vi "Manual.vi"() -> ()   [LabVIEW 2021]
uses:
  <vilib>/myRIO/Instrument Drivers/Onboard IO/DIO/typedefs/DIO Reference.ctl
  <vilib>/myRIO/Common/Instrument Driver Framework/Utilities/typedefs/myRIO Generic Hardware Reference.ctl
  <vilib>/myRIO/Common/Instrument Driver Framework/Utilities/typedefs/Hardware Version Enum.ctl
  <vilib>/myRIO/Common/Instrument Driver Framework/Utilities/typedefs/myRIO v1.0 Reference.ctl
  <vilib>/myRIO/Common/Instrument Driver Framework/Utilities/typedefs/Generic FPGA Reference.ctl
  <vilib>/myRIO/Common/Instrument Driver Framework/myRIO v1.0/DIO/typedefs/DIO Channels List.ctl
  <vilib>/myRIO/Common/Instrument Driver Framework/myRIO v1.0/DIO/typedefs/DIO Channels Enum.ctl
  <vilib>/userDefined/High Color/nirio_resource_hc.ctl
  <vilib>/myRIO/Instrument Drivers/Onboard IO/PWM/typedefs/PWM Reference.ctl
  <vilib>/myRIO/Common/Instrument Driver Framework/myRIO v1.0/PWM/typedefs/PWM Channels Enum.ctl
  <vilib>/myRIO/Instrument Drivers/Onboard IO/PWM/typedefs/PWM Configuration.ctl
  <vilib>/myRIO/Common/Instrument Driver Framework/Utilities/vis/Is FPGA Ref Available.vi
  <vilib>/myRIO/Common/Instrument Driver Framework/myRIO v1.0/DIO/vis/myRIO v1.1 Open DIO.vi
  <vilib>/myRIO/Instrument Drivers/Onboard IO/DIO/vis/Write.vi
  <vilib>/myRIO/Common/Instrument Driver Framework/myRIO v1.0/PWM/vis/myRIO v1.1 Open PWM.vi
  <vilib>/myRIO/Instrument Drivers/Onboard IO/PWM/vis/Set Duty Cycle and Frequency.vi
  <vilib>/myRIO/Common/Instrument Driver Framework/Utilities/vis/Validate Channels.vi
  <vilib>/myRIO/Common/Instrument Driver Framework/myRIO v1.0/DIO/vis/myRIO v1.0 Reserve DIO.vi
  <vilib>/myRIO/Common/Instrument Driver Framework/myRIO v1.0/PWM/vis/myRIO v1.0 Reserve PWM.vi
  <vilib>/myRIO/Common/Instrument Driver Framework/myRIO v1.0/Resource Manager/vis/myRIO v1.0 Reserve Channel List.vi
  <vilib>/myRIO/Common/Instrument Driver Framework/myRIO v1.0/DIO/vis/myRIO v1.0 Build MUX Configuration DIO.vi
  <vilib>/myRIO/Common/Instrument Driver Framework/myRIO v1.0/PWM/vis/myRIO v1.0 Build MUX Configuration PWM.vi
  <vilib>/myRIO/Common/Instrument Driver Framework/myRIO v1.0/Resource Manager/vis/myRIO v1.0 Reserve Channel.vi
  <vilib>/myRIO/Common/Instrument Driver Framework/myRIO v1.0/Resource Manager/vis/myRIO v1.0 Unreserve Channel.vi
  <vilib>/myRIO/Common/Instrument Driver Framework/myRIO v1.0/Resource Manager/vis/myRIO v1.0 Create Configuration List.vi
  <vilib>/myRIO/Common/Instrument Driver Framework/myRIO v1.0/Resource Manager/vis/myRIO v1.0 Build Mutex Name.vi
  <vilib>/Utility/VariantDataType/GetNumericInfo.vi
  <vilib>/Utility/error.llb/Error Cluster From Error Code.vi
  <vilib>/myRIO/Common/Instrument Driver Framework/myRIO v1.0/myRIO v1.1 Open.vi
  <vilib>/myRIO/Common/Instrument Driver Framework/Utilities/vis/IO Manager.vi
  <vilib>/myRIO/Common/Instrument Driver Framework/Utilities/vis/Configuration Manager.vi
  <vilib>/myRIO/Common/Instrument Driver Framework/myRIO v1.0/Resource Manager/vis/myRIO v1.0 Configure IO.vi
  <vilib>/myRIO/Common/Instrument Driver Framework/myRIO v1.0/myRIO v1.0 Close.vi
  <vilib>/myRIO/Common/Instrument Driver Framework/myRIO v1.0/DIO/vis/myRIO v1.0 Write DIO.vi
  <vilib>/myRIO/Common/Instrument Driver Framework/myRIO v1.0/PWM/vis/myRIO v1.0 Write PWM.vi
  <vilib>/myRIO/Express VI/Onboard IO/DO/DO Express VI.xnode
  <vilib>/myRIO/Instrument Drivers/Onboard IO/DIO/vis/myRIO DIO Open.xnode
  <vilib>/myRIO/Express VI/Onboard IO/PWM/PWM Express VI.xnode
  <vilib>/myRIO/Instrument Drivers/Onboard IO/PWM/vis/myRIO PWM Open.xnode
  <vilib>/myRIO/Instrument Drivers/Onboard IO/PWM/PWM.lvlib
  <vilib>/myRIO/Instrument Drivers/Onboard IO/DIO/DIO.lvlib
panel:
  out "Shoot Speed":dbl
  out "B":bool
  out "D":bool
  out "A":bool
  out "C":bool
  out "Robot Speed":dbl format="%#_1f"
  out "Joystick Status":bool
  out "Direction":dbl
  in  "stop":bool
  # "MOTOR ORIENTATION"
  # "MyRIO-SooYewGuan\n\n0.025\n0.125\n\n0.105\n0.125"
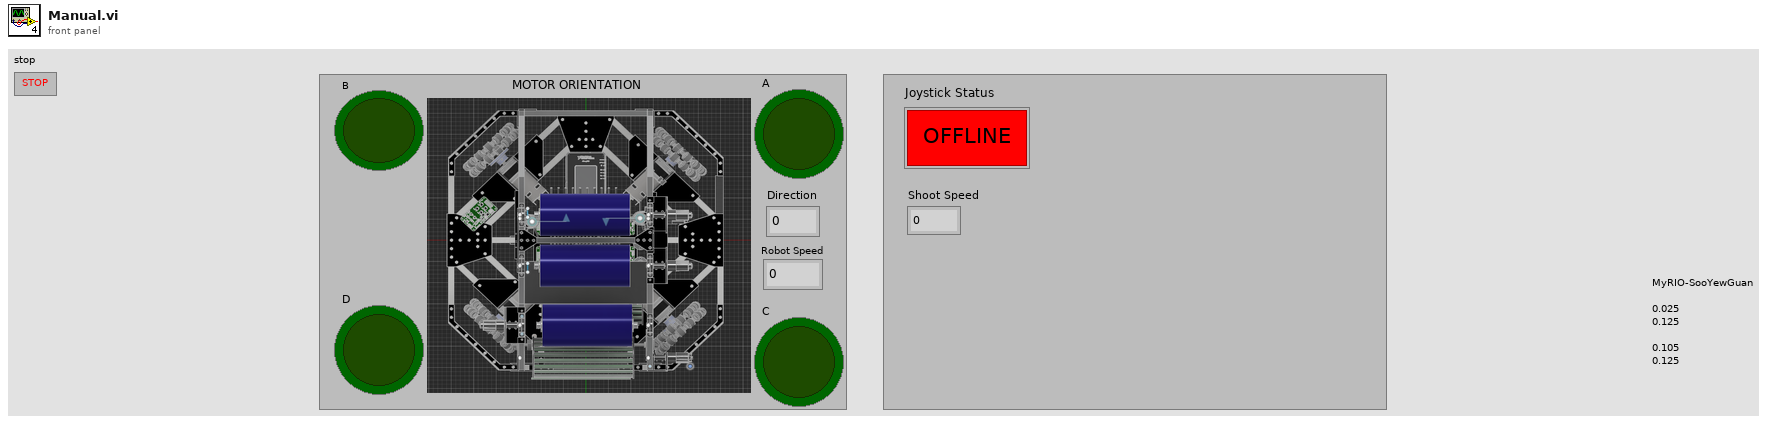
[diagram p1: front panel]
types:
  T1 = typedef "DIO.lvlib/DIO Reference.ctl" = cluster{"myRIO Reference":T2, "DIO Channels List":T6}
  T2 = typedef "myRIO Generic Hardware Reference.ctl" = cluster{"myRIO Model":T3, "myRIO Hardware Reference":T4}
  T3 = typedef "Hardware Version Enum.ctl" = enum16{"Unknown", "myRIO-1900", "myRIO-1950", "roboRIO", "NI ELVIS RIO CM", "ELVIS III"}
  T4 = typedef "myRIO v1.0 Reference.ctl" = cluster{"Generic FPGA Reference":T5, "Allow multiple opens":bool}
  T5 = typedef "Generic FPGA Reference.ctl" = refnum<k20>
  T6 = typedef "DIO Channels List.ctl" = T7[]
  T7 = typedef "DIO Channels Enum.ctl" = enum16{"Not Connected", "C/DIO0", "C/DIO1", "C/DIO2", "C/DIO3", "C/DIO4", "C/DIO5", "C/DIO6", "C/DIO7", "A/DIO0", "A/DIO1", "A/DIO2", "A/DIO3", "A/DIO4", "A/DIO5", "A/DIO6", "A/DIO7", "A/DIO8", "A/DIO9", "A/DIO10", "A/DIO11", "A/DIO12", "A/DIO13", "A/DIO14", "A/DIO15", "A/DIO16", "A/DIO17", "A/DIO18", "A/DIO19", "B/DIO0", "B/DIO1", "B/DIO2", "B/DIO3", "B/DIO4", "B/DIO5", "B/DIO6", "B/DIO7", "B/DIO8", "B/DIO9", "B/DIO10", "B/DIO11", "B/DIO12", "B/DIO13", "B/DIO14", "B/DIO15", "B/DIO16", "B/DIO17", "B/DIO18", "B/DIO19", "LED0", "LED1", "LED2", "LED3", "Button0", "DIO/DIO0", "DIO/DIO1", "DIO/DIO2", "DIO/DIO3", "DIO/DIO4", "DIO/DIO5", "DIO/DIO6", "DIO/DIO7", "DIO/DIO8", "DIO/DIO9", "SPI/CS0", "SPI/CS1", "SPI/CS2", "SPI/CS3", "LED RADIO (Green)", "LED RADIO (Red)", "LED COMM (Green)", "LED COMM (Red)", "LED MODE (Green)", "LED MODE (Red)"}
  T8 = typedef "nirio_resource_hc.ctl" = tag
  T9 = typedef "PWM.lvlib/PWM Reference.ctl" = cluster{"myRIO Reference":T2, "PWM Channels Enum":T10, "PWM Configuration":T11}
  T10 = typedef "PWM Channels Enum.ctl" = enum16{"Not Connected", "C/PWM0", "C/PWM1", "A/PWM0", "A/PWM1", "A/PWM2", "A/PWM3", "A/PWM4", "A/PWM5", "A/PWM6", "A/PWM7", "A/PWM8", "A/PWM9", "A/PWM10", "A/PWM11", "A/PWM12", "A/PWM13", "A/PWM14", "A/PWM15", "A/PWM16", "A/PWM17", "A/PWM18", "A/PWM19", "B/PWM0", "B/PWM1", "B/PWM2", "B/PWM3", "B/PWM4", "B/PWM5", "B/PWM6", "B/PWM7", "B/PWM8", "B/PWM9", "B/PWM10", "B/PWM11", "B/PWM12", "B/PWM13", "B/PWM14", "B/PWM15", "B/PWM16", "B/PWM17", "B/PWM18", "B/PWM19", "PWM/PWM0", "PWM/PWM1", "PWM/PWM2", "PWM/PWM3", "PWM/PWM4", "PWM/PWM5", "PWM/PWM6", "PWM/PWM7", "PWM/PWM8", "PWM/PWM9"}
  T11 = typedef "PWM.lvlib/PWM Configuration.ctl" = cluster{"Frequency":dbl, "Duty Cycle":dbl}
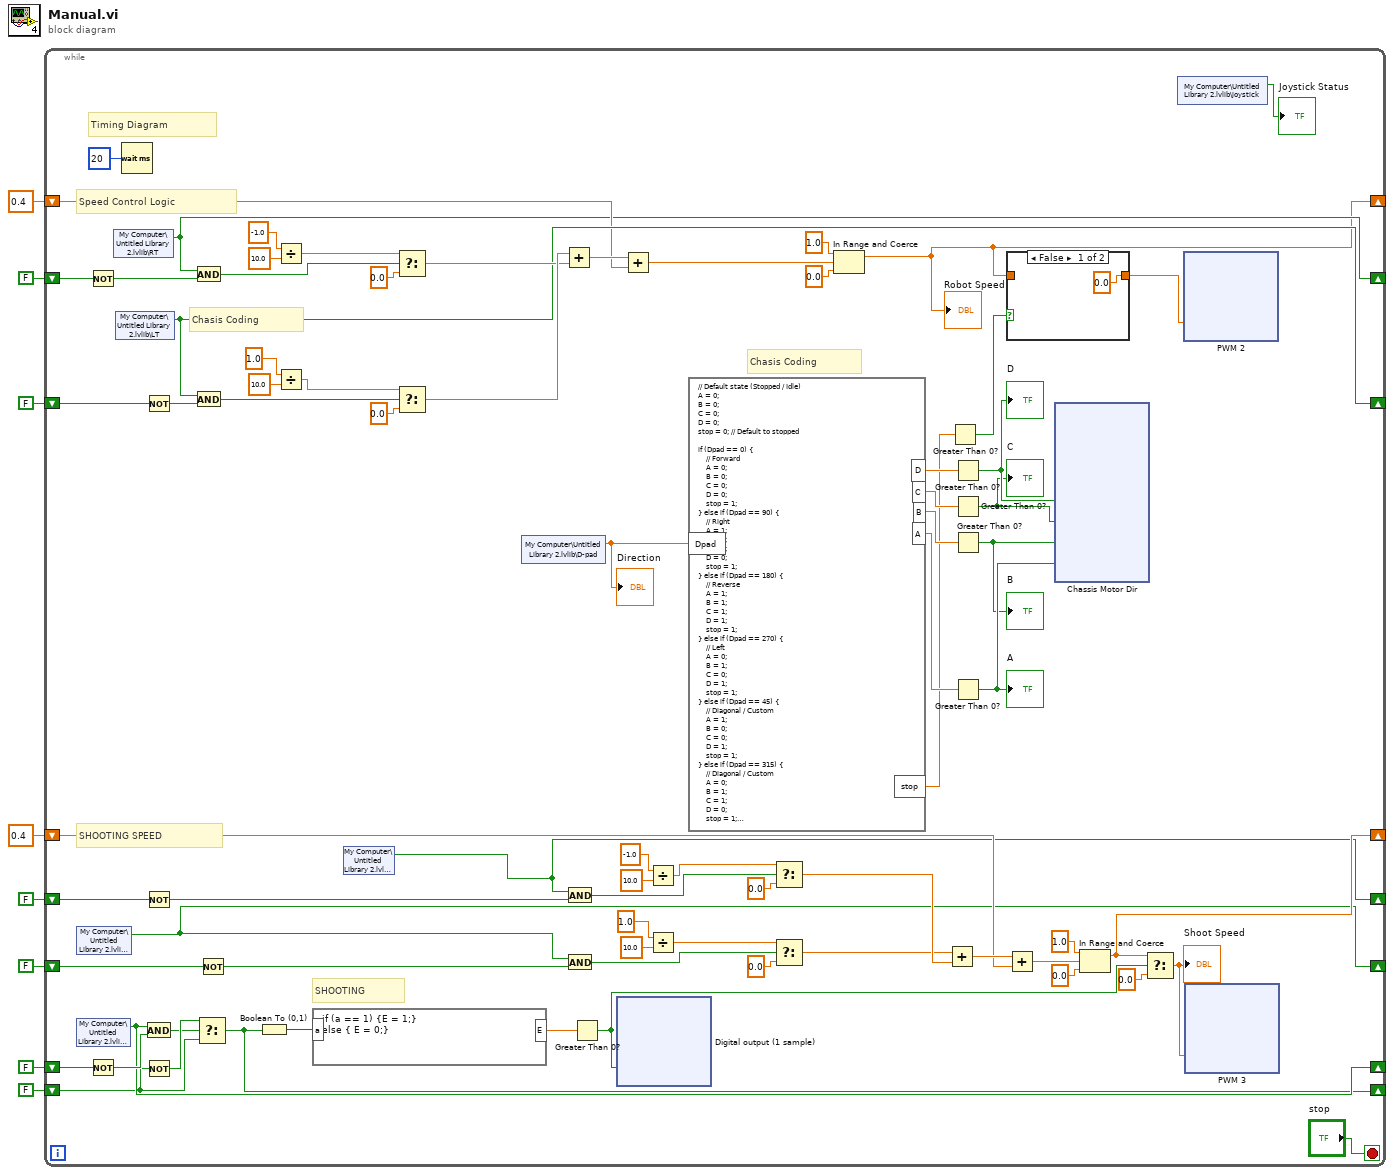
[diagram p0: block diagram]
diagram:
  n1 = while {
    shift-right: [w33] -> _
    shift-left: 0.4 ("Duty Cycle") -> [w53]
    shift-right: [w52] -> _
    shift-left: FALSE -> [w54]
    shift-right: [w55] -> _
    shift-left: FALSE -> [w56]
    shift-right: [w39] -> _
    shift-left: FALSE -> [w41]
    shift-right: [w34] -> _
    shift-left: FALSE -> [w37]
    shift-right: [w11] -> _
    shift-left: 0.4 ("Duty Cycle") -> [w14]
    shift-right: [w9] -> _
    shift-left: FALSE -> [w13]
    shift-right: [w10] -> _
    shift-left: FALSE -> [w12]
    stop <- "stop" stop-if-true
    # "Chasis Coding"
    # "SHOOTING SPEED"
    # "SHOOTING"
    # "Chasis Coding"
    # "Speed Control Logic"
    # "Timing Diagram"
    n2 = shared-variable "My Computer\\Untitled Library 2.lvlib\\+"() -> (w10:bool)  [unwired: 1 in, 1 out]
    n3 = shared-variable "My Computer\\Untitled Library 2.lvlib\\A"() -> (w39:bool)  [unwired: 1 in, 1 out]
    n4 = Not(x=w54) -> (.not. x?=w67:bool)
    n5 = Not(x=w41) -> (.not. x?=w40:bool)
    n6 = shared-variable "My Computer\\Untitled Library 2.lvlib\\RT"() -> (w52:bool)  [unwired: 1 in, 1 out]
    n7 = shared-variable "My Computer\\Untitled Library 2.lvlib\\LT"() -> (w55:bool)  [unwired: 1 in, 1 out]
    n8 = Wait (ms)(milliseconds to wait=u32 20) -> ()  [unwired: 1 out]
    n9 = Not(x=w56) -> (.not. x?=w74:bool)
    n10 = Not(x=w13) -> (.not. x?=w27:bool)
    n11 = And(x=w39, y=w40) -> (x .and. y?=w36:bool)
    n12 = Not(x=w37) -> (.not. x?=w38:bool)
    n13 = And(x=w52, y=w67) -> (x .and. y?=w62:bool)
    n14 = And(x=w55, y=w74) -> (x .and. y?=w73:bool)
    n15 = Select(t=w38, s=w36, f=w37) -> (s? t:f=w34:bool)
    n16 = Not(x=w12) -> (.not. x?=w23:bool)
    n17 = Boolean To (0,1)(Boolean=w34) -> (0, 1=w35:i16)
    n18 = Divide(x=-1.0, y=10.0) -> (x/y=w66:dbl)
    n19 = Divide(x=1.0, y=10.0) -> (x/y=w72:dbl)
    n20 = formula code="if (a == 1) {E = 1;} \nelse { E = 0;}"("a"=w35) -> ("E"=w43:dbl)
    n21 = shared-variable "My Computer\\Untitled Library 2.lvlib\\-"() -> (w9:bool)  [unwired: 1 in, 1 out]
    n22 = Select(t=w66, s=w62, f=0.0) -> (s? t:f=w60:dbl)
    n23 = Select(t=w72, s=w73, f=0.0) -> (s? t:f=w68:dbl)
    n24 = shared-variable "My Computer\\Untitled Library 2.lvlib\\D-pad"() -> (w76:dbl)  [unwired: 1 in, 1 out]
    "Direction" <- w76
    n25 = Add(x=w68, y=w60) -> (x+y=w61:dbl)
    n26 = And(x=w9, y=w27) -> (x .and. y?=w29:bool)
    n27 = And(x=w10, y=w23) -> (x .and. y?=w24:bool)
    n28 = Greater Than 0?(x=w43) -> (x > 0?=w42:bool)
    n29 = xnode "Digital output (1 sample)"("A/DIO0 (Pin 11)"=w42) -> ()  [unwired: 1 in, 1 out]
    n30 = Add(x=w61, y=w53) -> (x+y=w57:dbl)
    n31 = Divide(x=-1.0, y=10.0) -> (x/y=w28:dbl)
    n32 = Divide(x=1.0, y=10.0) -> (x/y=w25:dbl)
    n33 = formula code="// Default state (Stopped / Idle)\nA = 0;\nB = 0;\nC = 0;\nD = 0;\nstop = 0; // Default to stopped\n\nif (Dpad == 0) {\n    // Forward\n    A = 0;\n    B = 0;\n    C = 0;\n    D = 0;\n    stop = 1;\n} else if (Dpad == 90) {\n    // Right\n    A = 1;\n    B = 0;\n    C = 1;\n    D = 0;\n    stop = 1;\n} else if (Dpad == 180) {\n    // Reverse\n    A = 1;\n    B = 1;\n    C = 1;\n    D = 1;\n    stop = 1;\n} else if (Dpad == 270) {\n    // Left\n    A = 0;\n    B = 1;\n    C = 0;\n    D = 1;\n    stop = 1;\n} else if (Dpad == 45) {\n    // Diagonal / Custom\n    A = 1;\n    B = 0;\n    C = 0;\n    D = 1;\n    stop = 1;\n} else if (Dpad == 315) {\n    // Diagonal / Custom\n    A = 0;\n    B = 1;\n    C = 1;\n    D = 0;\n    stop = 1;\n}"("Dpad"=w76) -> ("A"=w82:dbl, "B"=w81:dbl, "C"=w80:dbl, "D"=w79:dbl, "stop"=w78:dbl)
    n34 = Select(t=w28, s=w29, f=0.0) -> (s? t:f=w31:dbl)
    n35 = Select(t=w25, s=w24, f=0.0) -> (s? t:f=w26:dbl)
    n36 = In Range and Coerce(upper limit=1.0, x=w57, lower limit=0.0) -> (coerced(x)=w33:dbl)  [unwired: 1 out]
    "Robot Speed" <- w33
    n37 = Add(x=w26, y=w31) -> (x+y=w30:dbl)
    n38 = Greater Than 0?(x=w78) -> (x > 0?=w77:bool)
    n39 = Greater Than 0?(x=w79) -> (x > 0?=w47:bool)
    "D" <- w47
    n40 = Greater Than 0?(x=w80) -> (x > 0?=w46:bool)
    "C" <- w46
    n41 = Greater Than 0?(x=w81) -> (x > 0?=w44:bool)
    "B" <- w44
    n42 = Greater Than 0?(x=w82) -> (x > 0?=w45:bool)
    "A" <- w45
    n43 = case shown="False" w77 {
      tunnel: [0.0 ("Duty Cycle") w228] -> w50
      tunnel: w33 -> [_ w228]
      frame False {
      }
      frame True {
      }
    }
    n44 = Add(x=w30, y=w14) -> (x+y=w32:dbl)
    n45 = xnode "Chassis Motor Dir"("C/DIO3 (DIO3)"=w47, "C/DIO2 (DIO2)"=w46, "C/DIO1 (DIO1)"=w44, "C/DIO0 (DIO0)"=w45) -> ()  [unwired: 1 in, 1 out]
    n46 = In Range and Coerce(upper limit=1.0, x=w32, lower limit=0.0) -> (coerced(x)=w11:dbl)  [unwired: 1 out]
    n47 = Select(t=w11, s=w42, f=0.0) -> (s? t:f=w49:dbl)
    "Shoot Speed" <- w49
    n48 = shared-variable "My Computer\\Untitled Library 2.lvlib\\joystick"() -> (→"Joystick Status":bool)  [unwired: 1 in, 1 out]
    n49 = xnode "PWM 2"("Duty Cycle"=w50) -> ()  [unwired: 1 in, 1 out]
    n50 = xnode "PWM 3"("Duty Cycle"=w49) -> ()  [unwired: 1 in, 1 out]
  }
